vi "AlliGator Image Histogram Ctrl Refnums.vi"(8 "error in (no error)":errorcluster) -> (0 "error out":errorcluster, 3 "Image Histogram Ctrl Refnums":T1)   [LabVIEW 2021, in "AlliGator Image Histogram.lvlib"]
uses:
  AlliGator Image Histogram.lvlib
  AlliGator Image Histogram Control Refnums.ctl
  Histograms/Linear Histogram Options.ctl
  Histograms/Histogram Bin Option.ctl
  Histograms/Histogram Bin Position.ctl
  Globals, Variables, Constants/AlliGator Refnums List.ctl
  GUI/AlliGator GUI.lvlib
  Histograms/Histograms.lvlib
panel:
  # "see the License on the block diagram (Ctrl+E or Window:Show Block Diagram)"
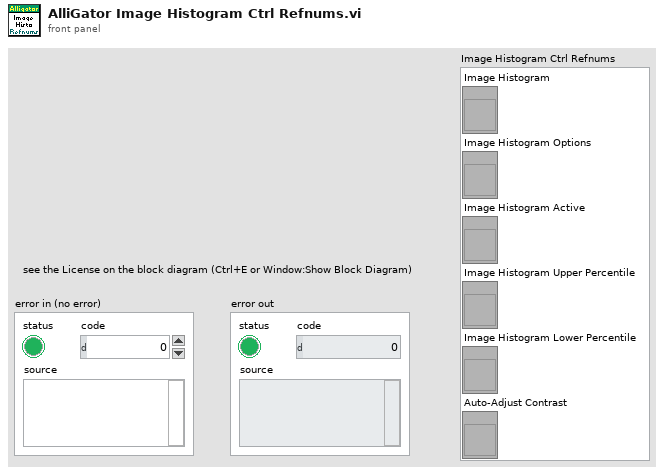
[diagram p1: front panel]
types:
  T1 = typedef "AlliGator Image Histogram.lvlib/AlliGator Image Histogram Control Refnums.ctl" = cluster{"Image Histogram":refnum<vi>, "Image Histogram Options":refnum<vi>, "Image Histogram Active":refnum<vi>, "Image Histogram Upper Percentile":refnum<vi>, "Image Histogram Lower Percentile":refnum<vi>, "Auto-Adjust Contrast":refnum<vi>}
  T2 = typedef "AlliGator GUI.lvlib/AlliGator Refnums List.ctl" = enum16{"---------- AlliGator Control Refnums ----------", "AlliGator Tab Control Refnum", "Dataset Ctrl Refnums", "Image Histogram Ctrl Refnums", "Intensity Time Trace Ctrl Refnums", "Decay Graph Ctrl Refnums", "Decay Statistics Graph Ctrl Refnums", "Phasor Graph Ctrl Refnums", "Phasor Ratio Graph Ctrl Refnums", "Phasor Plot Ctrl Refnums", "Lifetime & Other Parameters Ctrl Refnums", "Decay Fit Parameter Map Ctrl Refnums", "Parameter Map Ctrl Refnums", "Other AlliGator Ctrl Refnums", "---------- AlliGator Menu Refnums ----------", "AlliGator Menu", "---------- IO Device ID ----------", "Mouse ID", "Keyboard ID"}
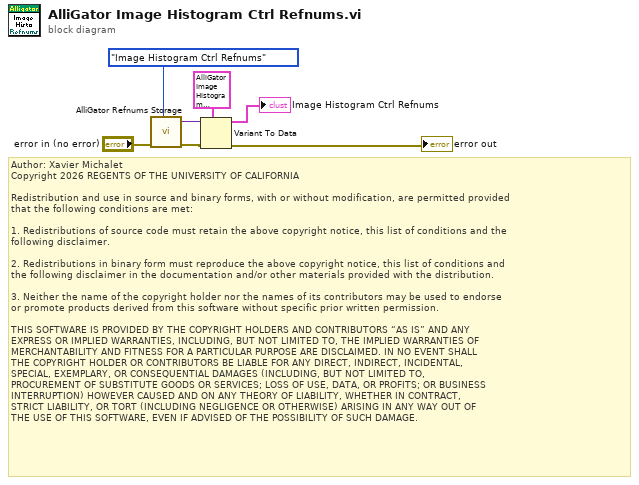
[diagram p0: block diagram]
diagram:
  # "Author: Xavier Michalet\nCopyright 2026 REGENTS OF THE UNIVERSITY OF CALIFORNIA\n\nRedistribution and use in source and binary forms, with or without modification, are permitted provided\nthat the following conditions are met:\n\n1. Redistributions of source code must retain the above copyright notice, this list of conditions and the\nfollowing disclaimer.\n\n2. Redistributions in binary form must reproduce the above copyright notice, this list of conditions and\nthe following disclaimer in the documentation and/or other materials provided with the distribution.\n\n3. Neither the name of the copyright holder nor the names of its contributors may be used to endorse \nor promote products derived from this software without specific prior written permission.\n\nTHIS SOFTWARE IS PROVIDED BY THE COPYRIGHT HOLDERS AND CONTRIBUTORS “AS IS” AND ANY \nEXPRESS OR IMPLIED WARRANTIES, INCLUDING, BUT NOT LIMITED TO, THE IMPLIED WARRANTIES OF\nMERCHANTABILITY AND FITNESS FOR A PARTICULAR PURPOSE ARE DISCLAIMED. IN NO EVENT SHALL\nTHE COPYRIGHT HOLDER OR CONTRIBUTORS BE LIABLE FOR ANY DIRECT, INDIRECT, INCIDENTAL, \nSPECIAL, EXEMPLARY, OR CONSEQUENTIAL DAMAGES (INCLUDING, BUT NOT LIMITED TO, \nPROCUREMENT OF SUBSTITUTE GOODS OR SERVICES; LOSS OF USE, DATA, OR PROFITS; OR BUSINESS\nINTERRUPTION) HOWEVER CAUSED AND ON ANY THEORY OF LIABILITY, WHETHER IN CONTRACT, \nSTRICT LIABILITY, OR TORT (INCLUDING NEGLIGENCE OR OTHERWISE) ARISING IN ANY WAY OUT OF\nTHE USE OF THIS SOFTWARE, EVEN IF ADVISED OF THE POSSIBILITY OF SUCH DAMAGE."
  n1 = call "AlliGator Refnums Storage.vi"("AlliGator Refnum List"=AlliGator_Refnums_List."Image Histogram Ctrl Refnums", "Error In"="error in (no error)") -> ("Error Out"=w2:errorcluster, "Data out"=w3:variant)  [unwired: 8 in]
  n2 = Variant To Data(error in=w2, type=T1 {"Image Histogram"=refnum, "Image Histogram Options"=refnum, "Image Histogram Active"=refnum, "Image Histogram Upper Percentile"=refnum, "Image Histogram Lower Percentile"=refnum, "Auto-Adjust Contrast"=refnum} ("Image Histogram Ctrl Refnums"), Variant=w3) -> (data=→"Image Histogram Ctrl Refnums":T1, error out=→"error out":errorcluster)
